vi "VIH - CHM Project - Write TOC File - Add TOC Record.vi"(5 "Project Files":T3, 6 "Level":i32, 7 "Base Dir Path":path, 10 "File Params":T2, 11 "HTML in":string) -> (3 "HTML out":string)   [LabVIEW 2014]
doc: "::: VI Helpeks :::\nCopyright (c) 2000-2026 Konstantin Shifershteyn. All rights reserved."
uses:
  _VIH HelpGen - Palette.llb/VIH HelpGen Typedef - Palette - Item Type Enum.ctl
panel:
  # "VI Helpeks\nCopyright (c) 2012-2026 Konstantin Shifershteyn"
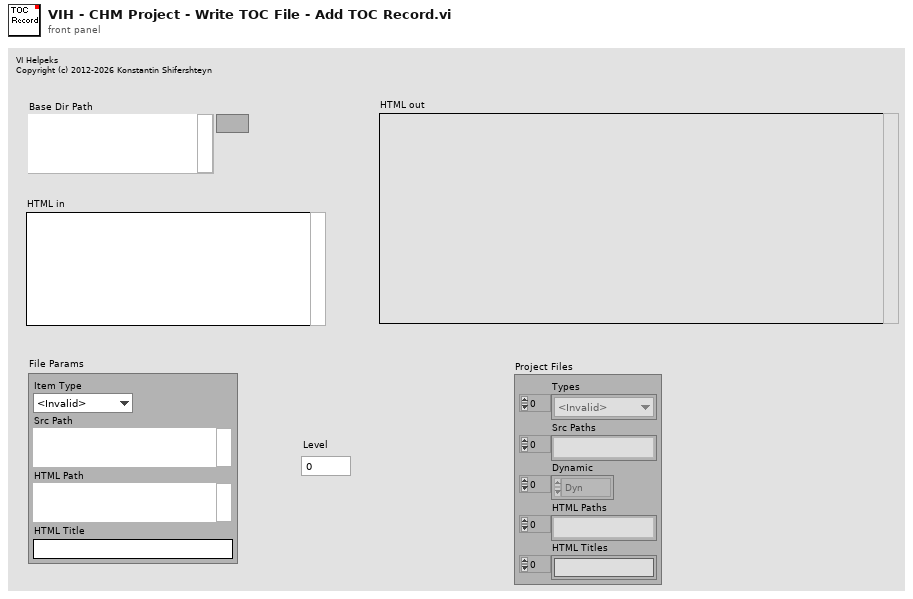
[diagram p1: front panel]
types:
  T1 = typedef "VIH HelpGen Typedef - Palette - Item Type Enum.ctl" = enum32{"<Invalid>", "<unknown>", "VI", "Menu", "LV Func", "Express VI", "Poly VI", "CTL", "HTML"}
  T2 = cluster{"Item Type":T1, "Src Path":path, "HTML Path":path, "HTML Title":string}
  T3 = cluster{"Types":T1[], "Src Paths":path[], "Dynamic":enum16{"Dyn", "Stat", "Both"}[], "HTML Paths":path[], "HTML Titles":string[]}
  T4 = cluster{"Item Type":T1, "Item File":path, "HTML File":path, "HTML Title":string}[]
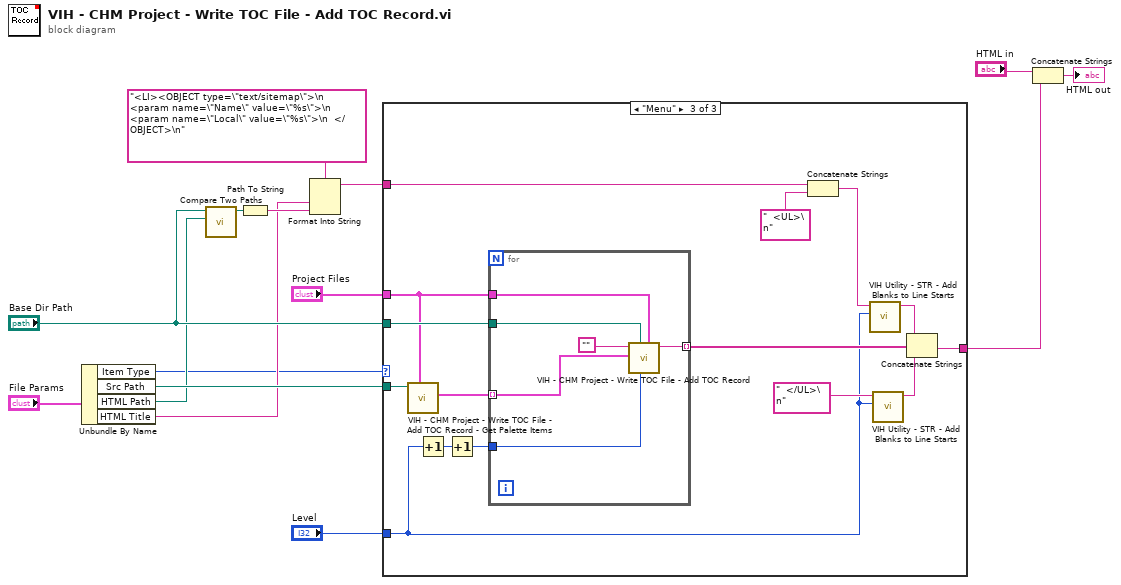
[diagram p0: block diagram]
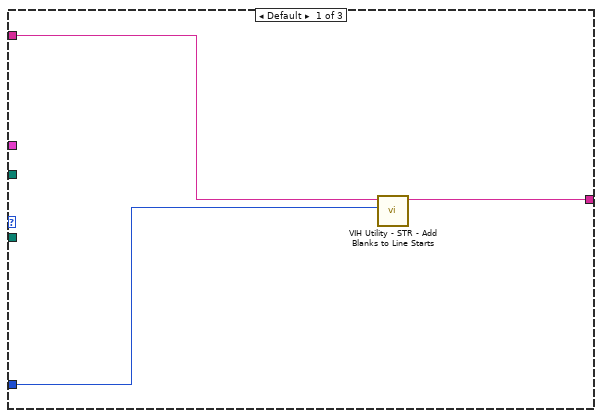
[diagram p2: hidden frame]
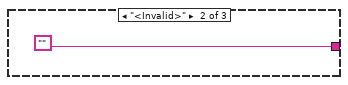
[diagram p3: hidden frame]
diagram:
  n1 = Unbundle By Name("File Params") -> ("Item Type"=w2:T1, "Src Path"=w7:path, "HTML Path"=w5:path, "HTML Title"=w6:string)
  n2 = call <vilib>:"Compare Two Paths.vi"("Path 2"=w5, "Path 1"="Base Dir Path") -> ("Relative Path from 1 to 2"=w14:path)  [unwired: 6 in, 3 out]
  n3 = Path To String(path=w14) -> (string=w13:string)
  n4 = Format Into String(format string="<LI><OBJECT type=\"text/sitemap\">\n  <param name=\"Name\" value=\"%s\">\n  <param name=\"Local\" value=\"%s\">\n  </OBJECT>\n", w6, w13) -> (resulting string=w12:string)  [unwired: 2 in, 1 out]
  n5 = case shown="\"Menu\"" w2 {
    tunnel: w12 -> [w18 _ w27]
    tunnel: [w16 "" w33] -> w3
    tunnel: w7 -> [_ _ w25]
    tunnel: "Base Dir Path" -> [_ _ w34]
    tunnel: "Project Files" -> [_ _ w24]
    tunnel: "Level" -> [w17 _ w22]
    frame Default {
      n6 = call "VIH Utility - STR - Add Blanks to Line Starts.vi"("level"=w17, "String"=w18) -> ("String out"=w16:string)  [unwired: 9 in]
    }
    frame "<Invalid>" {
    }
    frame "Menu" {
      n7 = call "VIH - CHM Project - Write TOC File - Add TOC Record - Get Palette Items.vi"("Project Files"=w24, "Palette Menu Path"=w25) -> ("Items"=w23:T4)  [unwired: 7 in, 2 out]
      n8 = Increment(x=w22) -> (x+1=w20:i32)
      n9 = Increment(x=w20) -> (x+1=w21:i32)
      n10 = for {
        tunnel: w34 -> [w40]
        tunnel: w24 -> [w39]
        tunnel: w21 -> [w35]
        tunnel: [w38] -> w32 mode=indexing
        tunnel: w23 -> [w36] mode=indexing
        n11 = call "VIH - CHM Project - Write TOC File - Add TOC Record.vi"("Project Files"=w39, "Level"=w35, "Base Dir Path"=w40, "File Params"=w36, "HTML in"="") -> ("HTML out"=w38:string)  [unwired: 6 in]
      }
      n12 = Concatenate Strings(w27, "  <UL>\n") -> (w29:string)
      n13 = call "VIH Utility - STR - Add Blanks to Line Starts.vi"("level"=w22, "String"=w29) -> ("String out"=w28:string)  [unwired: 9 in]
      n14 = call "VIH Utility - STR - Add Blanks to Line Starts.vi"("level"=w22, "String"="  </UL>\n") -> ("String out"=w30:string)  [unwired: 9 in]
      n15 = Concatenate Strings(w28, w32, w30) -> (w33:string)
    }
  }
  n16 = Concatenate Strings("HTML in", w3) -> (→"HTML out":string)
